vi "refresh.vi"(8 "error in":errorcluster, 10 "Engine Configuration In":refnum<class "engine configuration.lvclass">, 11 "Shared Memory editor node In":refnum<class "Shared Memory editor node.lvclass">) -> (0 "error out":errorcluster, 2 "Engine Configuration Out":refnum<class "engine configuration.lvclass">, 3 "Shared Memory editor node Out":refnum<class "Shared Memory editor node.lvclass">)   [LabVIEW 2014, in "Shared Memory editor node.lvclass"]
uses:
  Shared Memory editor node.lvclass
  <vilib>/NI/Module Execution Interface/Engine Configuration/engine configuration.lvclass
  <vilib>/NI/Configuration Framework/serializable configuration/get alias.vi
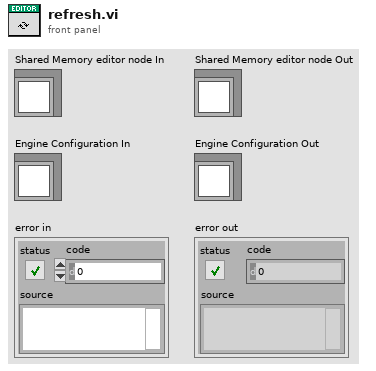
[diagram p1: front panel]
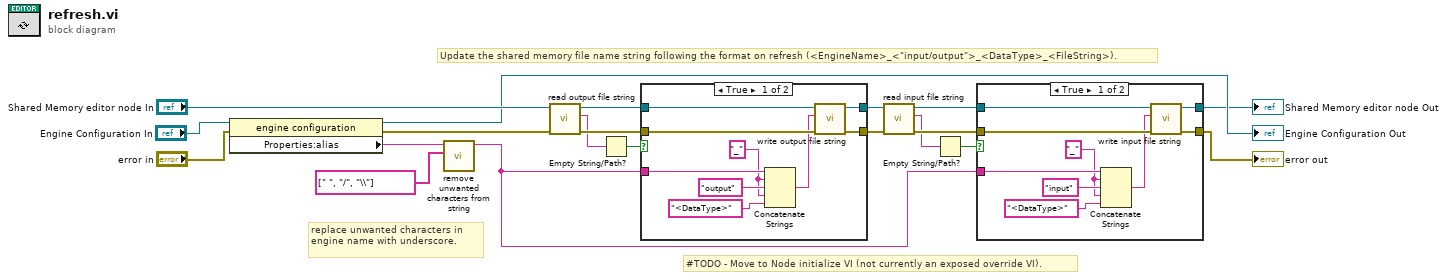
[diagram p0: block diagram]
diagram:
  # "replace unwanted characters in engine name with underscore."
  # "#TODO - Move to Node initialize VI (not currently an exposed override VI)."
  # "Update the shared memory file name string following the format on refresh (<EngineName>_<\"input/output\">_<DataType>_<FileString>)."
  n1 = property class="engine configuration"(reference="Engine Configuration In", error in="error in") -> (reference out=→"Engine Configuration Out":refnum<class "engine configuration.lvclass">, error out=w16:errorcluster, "Properties:alias"=w2:string)
  n2 = call "remove unwanted characters from string.vi"("unwanted patterns/characters"=string[] [" ", "/", "\\"], "string in"=w2) -> ("string out"=w3:string)  [unwired: 9 in]
  n3 = call "read output file string.vi"("error in"=w16, "shared memory editor node"="Shared Memory editor node In") -> ("error out"=w14:errorcluster, "output file string"=w5:string, "shared memory editor node out"=w15:refnum<class "Shared Memory editor node.lvclass">)  [unwired: 7 in]
  n4 = Empty String/Path?(string/path=w5) -> (empty?=w17:bool)
  n5 = case shown="True" w17 {
    tunnel: w3 -> [w25 _]
    tunnel: w15 -> [w29 w31]
    tunnel: w14 -> [w28 w30]
    tunnel: [w27 w31] -> w13
    tunnel: [w26 w30] -> w12
    frame True {
      w21 = "_" ("string")
      n6 = Concatenate Strings(w25, w21, "output", w21, "<DataType>") -> (w23:string)
      n7 = call "write output file string.vi"("error in"=w28, "output file string"=w23, "shared memory editor node"=w29) -> ("error out"=w26:errorcluster, "shared memory editor node out"=w27:refnum<class "Shared Memory editor node.lvclass">)  [unwired: 7 in]
    }
    frame False {
    }
  }
  n8 = call "read input file string.vi"("error in"=w12, "shared memory editor node"=w13) -> ("error out"=w20:errorcluster, "input file string"=w4:string, "shared memory editor node out"=w19:refnum<class "Shared Memory editor node.lvclass">)  [unwired: 7 in]
  n9 = Empty String/Path?(string/path=w4) -> (empty?=w18:bool)
  n10 = case shown="True" w18 {
    tunnel: w3 -> [w36 _]
    tunnel: w19 -> [w40 w42]
    tunnel: w20 -> [w39 w41]
    tunnel: [w38 w42] -> w7
    tunnel: [w37 w41] -> w6
    frame True {
      w32 = "_" ("string")
      n11 = Concatenate Strings(w36, w32, "input", w32, "<DataType>") -> (w34:string)
      n12 = call "write input file string.vi"("error in"=w39, "input file string"=w34, "shared memory editor node"=w40) -> ("error out"=w37:errorcluster, "shared memory editor node out"=w38:refnum<class "Shared Memory editor node.lvclass">)  [unwired: 7 in]
    }
    frame False {
    }
  }
  "Shared Memory editor node Out" <- w7
  "error out" <- w6
